vi "Get Map Values Array.vi"(0 "DBMap in":refnum<class "DBMap.lvclass">, 11 "error in (no error)":errorcluster {"code" format="Error %.0f"}) -> (4 "DBMap out":refnum<class "DBMap.lvclass">, 6 "File Data Array":T1[](array[typedef]), 15 "error out":errorcluster {"code" format="Error %.0f"})   [LabVIEW 2020, in "DBMap.lvclass"]
uses:
  DBMap.lvclass
  DBMap.lvclass/DBMap.ctl
  <vilib>/drjdpowell/SQLite Library/SQLite.lvlib
  <vilib>/drjdpowell/SQLite Library/SQL Connection/Execute SQL (1D String).vi
  <vilib>/drjdpowell/SQLite Library/SQL Connection/Connection.lvclass
  File Metadata.ctl
  Node.ctl
  Source to Sink Array.ctl
  File Data.ctl
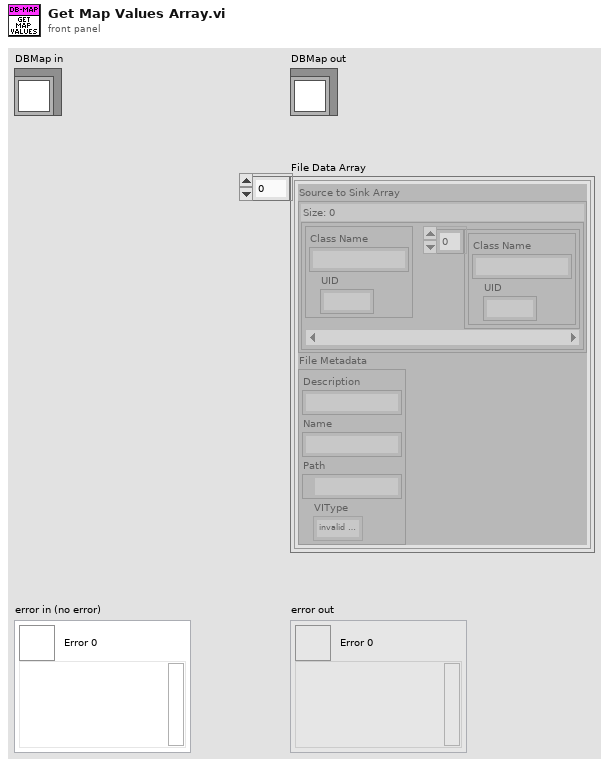
[diagram p1: front panel]
types:
  T1 = typedef "File Data.ctl" = cluster{"Source to Sink Array":T2, "File Metadata":T4}
  T2 = typedef "Source to Sink Array.ctl" = map{T3, T3[]}
  T3 = typedef "Node.ctl" = cluster{"Class Name":string, "UID":i32}
  T4 = typedef "File Metadata.ctl" = cluster{"Description":string, "Name":string, "Path":path, "VIType":enum32{"invalid VI type", "Standard VI", "Control VI", "Global VI", "Polymorphic VI", "Configuration VI", "SubSystem", "Facade VI", "Method VI", "Statechart Diagram VI"}}
  T5 = typedef "Semaphore RefNum" = refnum<k1>
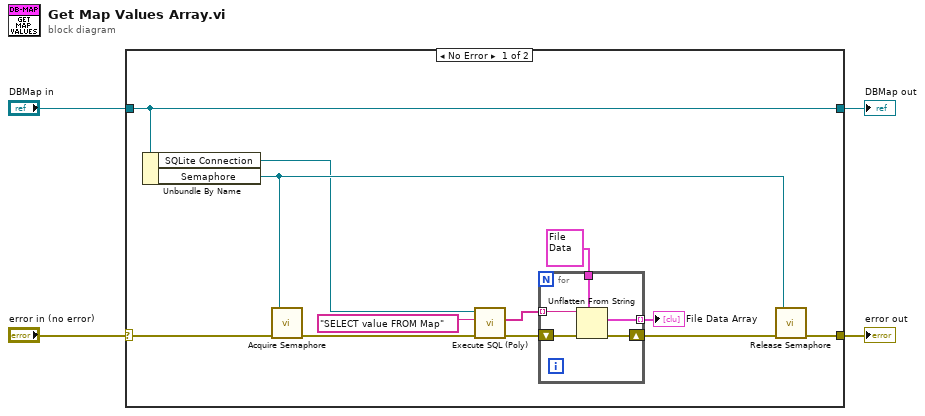
[diagram p0: block diagram]
diagram:
  n1 = case shown="No Error" "error in (no error)" {
    selector: "error in (no error)" -> [w15 w23]
    tunnel: [w14 w23] -> w3
    tunnel: [w16 w22] -> w1
    tunnel: "DBMap in" -> [w16 w22]
    frame No Error {
      n2 = Unbundle By Name(w16) -> ("SQLite Connection"=w7:refnum<class "Connection.lvclass">, "Semaphore"=w13:T5)
      n3 = call <vilib>:"Acquire Semaphore.vi"("error in (no error)"=w15, "semaphore"=w13) -> ("error out"=w9:errorcluster)  [unwired: 3 in, 2 out]
      n4 = call-poly <vilib>:"Execute SQL (Poly).vi"("error in (no error)"=w9, "SQL"="SELECT value FROM Map", "SQLite Connection in"=w7) -> ("error out"=w11:errorcluster, "Result Set"=w10:string[])  [unwired: 5 in, 2 out]
      n5 = for {
        shift-right: [w20] -> w8
        shift-left: w11 -> [w21]
        tunnel: T1 {"Source to Sink Array"={}, "File Metadata"={"Description"="", "Name"="", "Path"=path "", "VIType"=enum."invalid VI type"}} ("File Data") -> [w18]
        tunnel: w10 -> [w19] mode=indexing
        tunnel: [w17] -> w5 mode=indexing
        n6 = Unflatten From String(type=w18, binary string=w19, error in (no error)=w21) -> (value=w17:T1, error out=w20:errorcluster)  [unwired: 2 in, 1 out]
      }
      "File Data Array" <- w5
      n7 = call <vilib>:"Release Semaphore.vi"("error in (no error)"=w8, "semaphore"=w13) -> ("error out"=w14:errorcluster)  [unwired: 4 in, 1 out]
    }
    frame Error {
    }
  }
  "error out" <- w3
  "DBMap out" <- w1
